vi "GDM-9052 Read Dual Display.vi"() -> ()   [LabVIEW 2021, in "GDM-9052.lvlib"]
uses:
  GDM-9052.lvlib
panel:
  in  "2nd Function":u8(ring)=8 items=["DC Voltage", "AC Voltage", "DC Current", "AC Current", "2-Wire Resistance", "4-Wire Resistance", "Frequency", "Period", "None"]
  in  "1st Function":u8(ring) items=["DC Voltage", "AC Voltage", "DC Current", "AC Current", "2-Wire Resistance", "4-Wire Resistance", "Frequency", "Period", "Continuity", "Diode", "Temperature", "Capacitance"]
  in  "Manual Range":dbl format="%#.9e"
  in  "Manual Range":dbl format="%#.9e"
  in  "Configure RS232 Baud Rate":u32(ring)=115200 items=["9600"=9600, "19200"=19200, "38400"=38400, "57600"=57600, "115200"=115200]
  in  "Detector Rate":u8(ring) items=["SLOW", "MID", "FAST"]
  in  "Enable Auto Range":bool=TRUE
  in  "Enable Auto Range":bool=TRUE
  out "error out":errorcluster
  in  "Reset":bool
  out "Measure 2nd Value":string
  out "Measure 1st Value":string
  in  "Stop":bool
  out "Boolean":bool
  out "ID Return String":string
  in  "VISA resource name":refnum<visa-resource-name>
  # "GDM-9052 Dual Display"
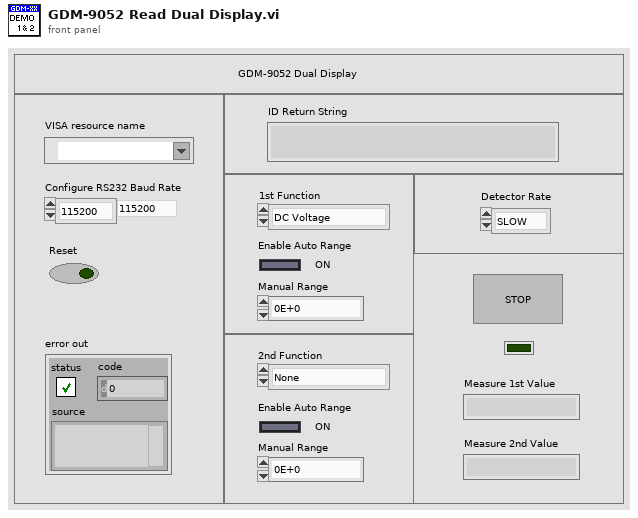
[diagram p1: front panel]
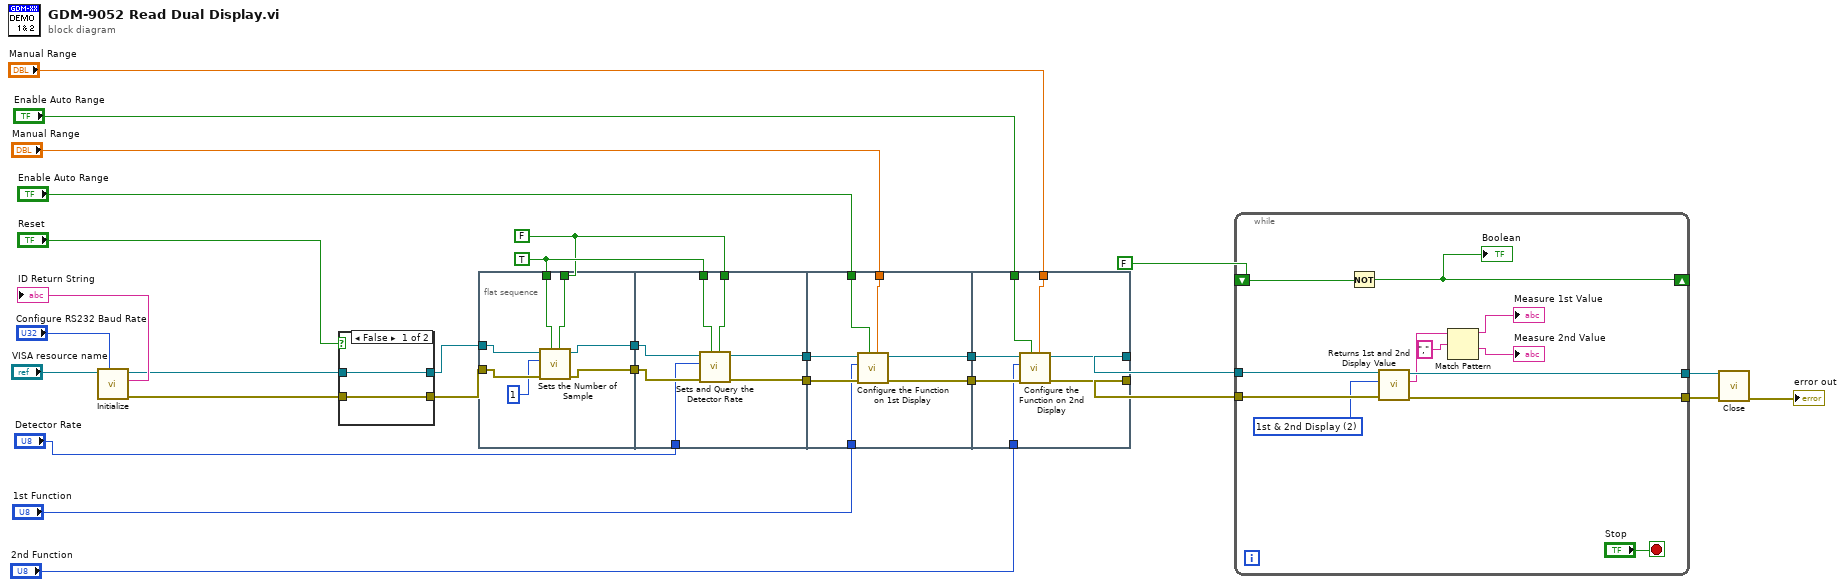
[diagram p0: block diagram]
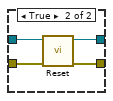
[diagram p2: hidden frame]
diagram:
  w8 = FALSE ("Enable to Query")
  w9 = TRUE ("Enable to Sets")
  n1 = call "Initialize.vi"("Configure RS232 Baud Rate"="Configure RS232 Baud Rate", "VISA resource name"="VISA resource name") -> ("error out"=w6:errorcluster, "ID Return String"=→"ID Return String":string, "VISA resource name out"=w7:refnum<visa-resource-name>)  [unwired: 6 in, 1 out]
  n2 = case shown="False" "Reset" {
    tunnel: [w31 w35] -> w20
    tunnel: [w30 w34] -> w19
    tunnel: w7 -> [w31 w33]
    tunnel: w6 -> [w30 w32]
    frame False {
    }
    frame True {
      n3 = call "Reset.vi"("error in (no error)"=w32, "VISA resource name"=w33) -> ("error out"=w34:errorcluster, "VISA resource name out"=w35:refnum<visa-resource-name>)  [unwired: 8 in]
    }
  }
  n4 = flat-sequence {
    tunnel: w19 -> [w39]
    tunnel: w20 -> [w42]
    tunnel: [w41] -> w11
    tunnel: [w40] -> w10
    tunnel: w9 -> [w37]
    tunnel: w8 -> [w36]
    tunnel: w8 -> [w49]
    tunnel: w9 -> [w48]
    tunnel: [w45] -> w16
    tunnel: [w44] -> w15
    tunnel: "Detector Rate" -> [w43]
    tunnel: w11 -> [w47]
    tunnel: w10 -> [w46]
    tunnel: "Enable Auto Range" -> [w56]
    tunnel: w16 -> [w55]
    tunnel: w15 -> [w54]
    tunnel: [w53] -> w14
    tunnel: [w52] -> w13
    tunnel: "Manual Range" -> [w51]
    tunnel: "1st Function" -> [w50]
    tunnel: [w60] -> w22
    tunnel: [w59] -> w21
    tunnel: "Enable Auto Range" -> [w63]
    tunnel: w14 -> [w62]
    tunnel: w13 -> [w61]
    tunnel: "Manual Range" -> [w58]
    tunnel: "2nd Function" -> [w57]
    frame #0 {
      n5 = call "Sets the Number of Sample.vi"("Enable to Query"=w36, "Enable to Sets"=w37, "error in"=w39, "Number of Sample"=u16 1, "VISA resource name"=w42) -> ("error out"=w40:errorcluster, "VISA resource name out"=w41:refnum<visa-resource-name>)  [unwired: 4 in, 1 out]
    }
    frame #1 {
      n6 = call "Sets and Query the Detector Rate.vi"("Enable to Query"=w49, "Enable to Sets"=w48, "error in"=w46, "Detector Rate"=w43, "VISA resource name"=w47) -> ("error out"=w44:errorcluster, "VISA resource name out"=w45:refnum<visa-resource-name>)  [unwired: 4 in, 1 out]
    }
    frame #2 {
      n7 = call "Configure the Function on 1st Display .vi"("Manual Range"=w51, "Enable Auto Range"=w56, "error in"=w54, "Function"=w50, "VISA resource name"=w55) -> ("error out"=w52:errorcluster, "VISA resource name out"=w53:refnum<visa-resource-name>)  [unwired: 5 in]
    }
    frame #3 {
      n8 = call "Configure the Function on 2nd Display.vi"("Manual Range"=w58, "Enable Auto Range"=w63, "error in"=w61, "Function"=w57, "VISA resource name"=w62) -> ("error out"=w59:errorcluster, "VISA resource name out"=w60:refnum<visa-resource-name>)  [unwired: 5 in]
    }
  }
  n9 = while {
    tunnel: w22 -> [w75]
    tunnel: w21 -> [w74]
    tunnel: [w72] -> w27
    tunnel: [w71] -> w26
    shift-right: [w69] -> _
    shift-left: FALSE -> [w70]
    stop <- "Stop" stop-if-true
    w66 = u16 2 items=["1st Display", "2nd Display", "1st & 2nd Display"] ("Sets to Display")
    n10 = Not(x=w70) -> (.not. x?=w69:bool)
    "Boolean" <- w69
    n11 = call "Returns 1st and 2nd Display Value.vi"("error in"=w74, "Sets to Display"=w66, "VISA resource name"=w75) -> ("error out"=w71:errorcluster, "Return the Value"=w68:string, "VISA resource name out"=w72:refnum<visa-resource-name>)  [unwired: 6 in]
    n12 = Match Pattern(string=w68, regular expression=",") -> (before substring=→"Measure 1st Value":string, after substring=→"Measure 2nd Value":string)  [unwired: 1 in, 2 out]
  }
  n13 = call "Close.vi"("error in (no error)"=w26, "VISA resource name"=w27) -> ("error out"=→"error out":errorcluster)  [unwired: 9 in]
